vi "根据点击位置找索引.vi"(1 "坐标":cluster{"水平":i32, "垂直":i32}, 2 "位置":cluster{"左":i32, "顶":i32}, 3 "边界":cluster{"宽":i32, "高":i32}) -> (0 "索引":i32)   [LabVIEW 2017]
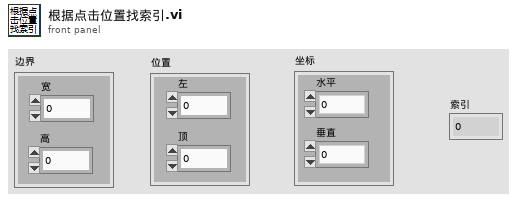
[diagram p1: front panel]
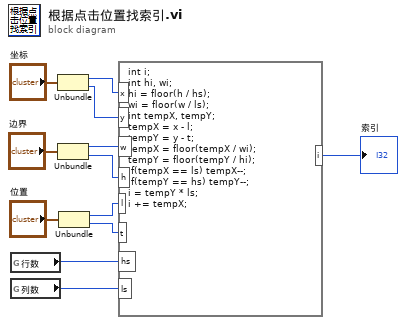
[diagram p0: block diagram]
diagram:
  n1 = global read "全局变量.vi" "行数"() -> (w2:i32)
  n2 = global read "全局变量.vi" "列数"() -> (w1:i32)
  n3 = Unbundle("坐标") -> ("水平"=w9:i32, "垂直"=w8:i32)
  n4 = Unbundle("边界") -> ("宽"=w7:i32, "高"=w6:i32)
  n5 = Unbundle("位置") -> ("左"=w5:i32, "顶"=w4:i32)
  n6 = formula code="int i;\nint hi, wi;\nhi = floor(h / hs);\nwi = floor(w / ls);\nint tempX, tempY;\ntempX = x - l;\ntempY = y - t;\ntempX = floor(tempX / wi);\ntempY = floor(tempY / hi);\nif(tempX == ls) tempX--;\nif(tempY == hs) tempY--;\ni = tempY * ls;\ni += tempX;"("x"=w9, "y"=w8, "l"=w5, "t"=w4, "w"=w7, "h"=w6, "hs"=w2, "ls"=w1) -> ("i"=→"索引":i32)
